vi "Read_Register.vi"(8 "error in (no error)":errorcluster, 9 "Quantity":u16, 10 "Start Address":u16, 11 "Modbus_Master in":refnum<class "Modbus_Master.lvclass">) -> (0 "error out":errorcluster, 2 "register values":u16[](array[numeric]), 3 "Modbus_Master out":refnum<class "Modbus_Master.lvclass">)   [LabVIEW 2021, in "Modbus_Master.lvclass"]
uses:
  Modbus_Master.lvclass
  Modbus_Master.lvclass/Modbus_Master.ctl
  <vilib>/NI/Modbus Library/API/Modbus API.lvclass/Modbus API.ctl
  <vilib>/NI/Modbus Library/Transmission Data Unit/Transmission Data Unit.lvclass/Transmission Data Unit.ctl
  <vilib>/NI/Modbus Library/Transmission Data Unit/Write Unit ID.vi
  <vilib>/NI/Modbus Library/API/Read Transmission Data Unit.vi
  <vilib>/NI/Modbus Library/API/Write Transmission Data Unit.vi
  <vilib>/NI/Modbus Library/API/Master/Modbus Master.lvclass
  C:/Program Files/National Instruments/LabVIEW 2021/vi.lib/NI/Modbus Library/API/Modbus API.lvclass
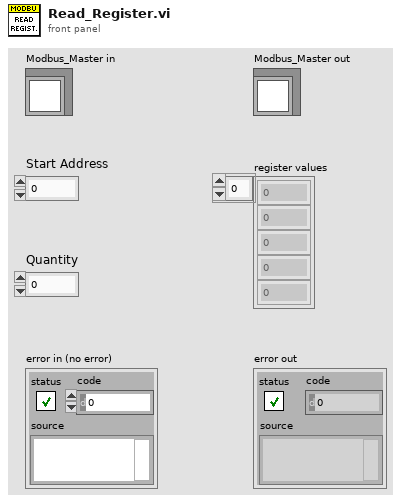
[diagram p1: front panel]
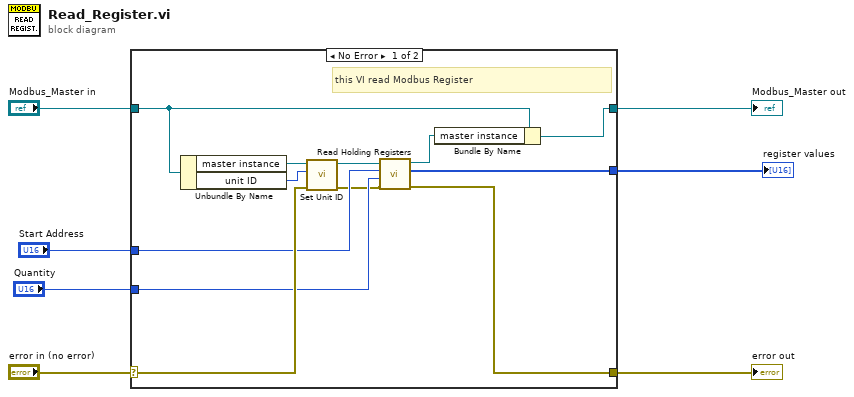
[diagram p0: block diagram]
diagram:
  n1 = case shown="No Error" "error in (no error)" {
    selector: "error in (no error)" -> [w17 w21]
    tunnel: [w12 w21] -> w6
    tunnel: [w8 w20] -> w4
    tunnel: "Modbus_Master in" -> [w9 w20]
    tunnel: "Start Address" -> [w15 _]
    tunnel: "Quantity" -> [w14 _]
    tunnel: [w11 _] -> w1
    frame No Error {
      # "this VI read Modbus Register"
      n2 = Unbundle By Name(w9) -> ("master instance"=w19:refnum<class "Modbus Master.lvclass">, "unit ID"=w18:u8)
      n3 = call <vilib>:"Set Unit ID.vi"("error in"=w17, "unit ID"=w18, "Modbus master in"=w19) -> ("error out"=w13:errorcluster, "Modbus master out"=w16:refnum<class "Modbus Master.lvclass">)  [unwired: 7 in]
      n4 = call-dynamic "Read Holding Registers.vi"("error in"=w13, "number of inputs"=w14, "starting address"=w15, "Modbus master in"=w16) -> ("error out"=w12:errorcluster, "register values"=w11:u16[], "Modbus master out"=w10:refnum<class "Modbus Master.lvclass">)  [unwired: 5 in]
      n5 = Bundle By Name(cluster=w9, "master instance"=w10) -> (w8:refnum<class "Modbus_Master.lvclass">)
    }
    frame Error {
    }
  }
  "error out" <- w6
  "Modbus_Master out" <- w4
  "register values" <- w1
